vi "Library Initialize and Exit.vi"(7 "action":enum16{"LibInit", "LibExit"}(ring), 8 "error in":errorcluster) -> (0 "error out":errorcluster, 1 "modules found":i32, 3 "instance count":i32)   [LabVIEW 2020, in "AIM ARINC 429 Hardware API.lvlib"]
uses:
  AIM ARINC 429 Hardware API.lvlib
  <instrlib>/AIM GmbH/_ARINC-429/AIM429LV.lvlib
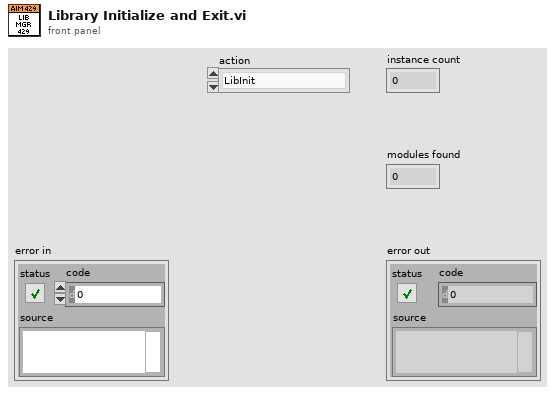
[diagram p1: front panel]
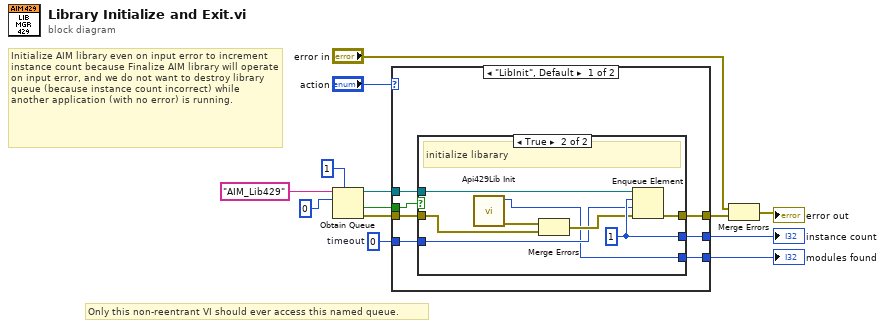
[diagram p0: block diagram]
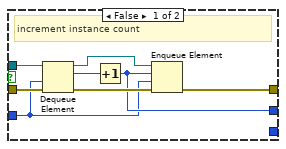
[diagram p2: hidden frame]
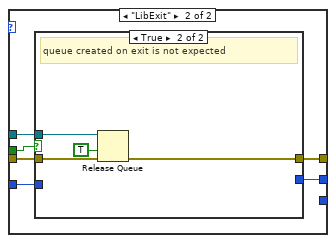
[diagram p3: hidden frame]
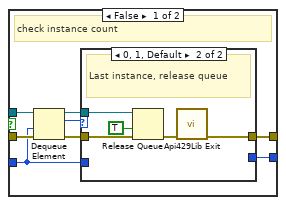
[diagram p4: hidden frame]
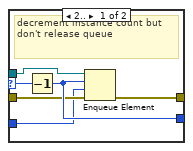
[diagram p5: hidden frame]
diagram:
  w1 = 0  # timeout
  # "Initialize AIM library even on input error to increment instance count because Finalize AIM library will operate on input error, and we do not want to destroy library queue (because instance count incorrect) while another application (with no error) is running."
  # "Only this non-reentrant VI should ever access this named queue."
  n1 = Obtain Queue(max queue size (-1, unlimited)=1, name (unnamed)="AIM_Lib429", element data type=0) -> (queue out=w4:refnum<queue>, created new?=w3:bool, error out=w2:errorcluster)  [unwired: 2 in]
  n2 = case shown="\"LibInit\", Default" "action" {
    tunnel: [w20 w42] -> w11
    tunnel: [w19 w41] -> w13
    tunnel: [w18 _] -> w12
    tunnel: w4 -> [w17 w40]
    tunnel: w3 -> [w16 w39]
    tunnel: w2 -> [w15 w38]
    tunnel: w1 -> [w14 w37]
    frame "LibInit", Default {
      n3 = case shown="True" w16 {
        tunnel: w15 -> [w27 w32]
        tunnel: [w24 w36] -> w20
        tunnel: [w23 w34] -> w19
        tunnel: w17 -> [w28 w35]
        tunnel: [_ w29] -> w18
        tunnel: w14 -> [w21 w31]
        frame False {
          # "increment instance count"
          n4 = Dequeue Element(queue=w28, timeout in ms (-1)=w21, error in (no error)=w27) -> (queue out=w26:refnum<queue>, element=w22:i32, error out=w25:errorcluster)  [unwired: 1 out]
          n5 = Increment(x=w22) -> (x+1=w23:i32)
          n6 = Enqueue Element(queue=w26, element=w23, timeout in ms (-1)=w21, error in (no error)=w25) -> (error out=w24:errorcluster)  [unwired: 2 out]
        }
        frame True {
          w34 = 1 ("modules found")
          # "initialize libarary"
          n7 = call <instrlib>:"Api429Lib Init.vi"() -> ("error out"=w30:errorcluster, "modules found"=w29:i32)  [unwired: 10 in]
          n8 = Merge Errors(w30, w32) -> (w33:errorcluster)
          n9 = Enqueue Element(queue=w35, element=w34, timeout in ms (-1)=w31, error in (no error)=w33) -> (error out=w36:errorcluster)  [unwired: 2 out]
        }
      }
    }
    frame "LibExit" {
      n10 = case shown="True" w39 {
        tunnel: [w50 w63] -> w42
        tunnel: [w49 _] -> w41
        tunnel: w40 -> [w48 w65]
        tunnel: w38 -> [w47 w64]
        tunnel: w37 -> [w43 _]
        frame False {
          # "check instance count"
          n11 = Dequeue Element(queue=w48, timeout in ms (-1)=w43, error in (no error)=w47) -> (queue out=w45:refnum<queue>, element=w46:i32, error out=w44:errorcluster)  [unwired: 1 out]
          n12 = case shown="0, 1, Default" w46 {
            selector: w46 -> [w54 _]
            tunnel: [w55 w58] -> w50
            tunnel: [w56 _] -> w49
            tunnel: w45 -> [w53 w61]
            tunnel: w44 -> [w52 w60]
            tunnel: w43 -> [w51 _]
            frame 2.. {
              # "decrement instance count but don't release queue"
              n13 = Decrement(x=w54) -> (x-1=w56:i32)
              n14 = Enqueue Element(queue=w53, element=w56, timeout in ms (-1)=w51, error in (no error)=w52) -> (error out=w55:errorcluster)  [unwired: 2 out]
            }
            frame 0, 1, Default {
              # "Last instance, release queue"
              n15 = Release Queue(queue=w61, force destroy? (F)=TRUE, error in (no error)=w60) -> (error out=w59:errorcluster)  [unwired: 2 out]
              n16 = call <instrlib>:"Api429Lib Exit.vi"("error in (no error)"=w59) -> ("error out"=w58:errorcluster)  [unwired: 10 in]
            }
          }
        }
        frame True {
          # "queue created on exit is not expected"
          n17 = Release Queue(queue=w65, force destroy? (F)=TRUE, error in (no error)=w64) -> (error out=w63:errorcluster)  [unwired: 2 out]
        }
      }
    }
  }
  "instance count" <- w13
  "modules found" <- w12
  n18 = Merge Errors("error in", w11) -> (→"error out":errorcluster)
